vi "ZM-ROOT-stop.vi"(8 "error in (no error)":errorcluster, 11 "ZM-ROOT-root in":refnum<class "ZM-ROOT-root.lvclass">) -> (0 "error out":errorcluster, 3 "ZM-ROOT-root out":refnum<class "ZM-ROOT-root.lvclass">)   [LabVIEW 2020, in "ZM-ROOT-root.lvlib" / "ZM-ROOT-root.lvclass"]
doc: "Stop hook of the root, called in Actor Core after Call Parent: fires the stop user event, so the event loop of ZM-ROOT-helperPanel ends. The error goes on to ZM-ROOT-close."
uses:
  ZM-ROOT-root.lvclass
  ZM-ROOT-root.lvclass/ZM-ROOT-root.ctl
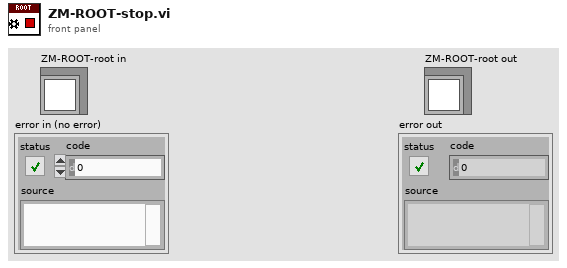
[diagram p1: front panel]
types:
  T1 = typedef "ZM-ROOT-root.lvlib/ZM-ROOT-root.lvclass/ZM-ROOT-EVENTS.ctl" = cluster{"stop":refnum<user-event>, "error":refnum<user-event>}
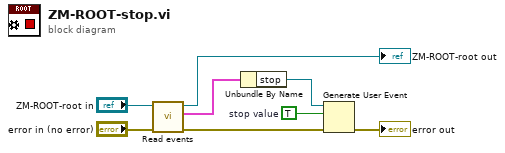
[diagram p0: block diagram]
diagram:
  w4 = TRUE  # stop value
  n1 = call "Read events.vi"("error in (no error)"="error in (no error)", "ZM-ROOT-root in"="ZM-ROOT-root in") -> ("error out"=w3:errorcluster, "ZM-ROOT-EVENTS"=w6:T1, "ZM-ROOT-root out"=→"ZM-ROOT-root out":refnum<class "ZM-ROOT-root.lvclass">)  [unwired: 7 in]
  n2 = Unbundle By Name(w6) -> ("stop"=w5:refnum<user-event>)
  n3 = Generate User Event(user event=w5, event data cluster=w4, error in=w3) -> (error out=→"error out":errorcluster)  [unwired: 1 in, 1 out]
